vi "Driver_Event.vi"(0 "Data":variant, 2 "Event":T1, 11 "Error In":errorcluster, 13 "Event Operation":T2) -> (4 "Event Ref":refnum<user-event>, 15 "Error Out":errorcluster)   [LabVIEW 2026, in "Core.lvlib"]
doc: "Event driver for all the events in the project."
uses:
  Core.lvlib
  TypeDefs/Enum_Event_Options.ctl
  TypeDefs/Enum_Events.ctl
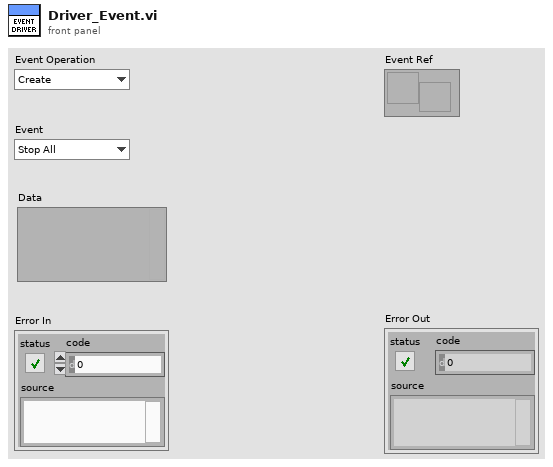
[diagram p1: front panel]
types:
  T1 = typedef "Core.lvlib/Enum_Events.ctl" = enum16{"Stop All", "Stop SubVI", "Update Object"}
  T2 = typedef "Core.lvlib/Enum_Event_Options.ctl" = enum16{"Create", "Generate", "Event Ref", "Destroy"}
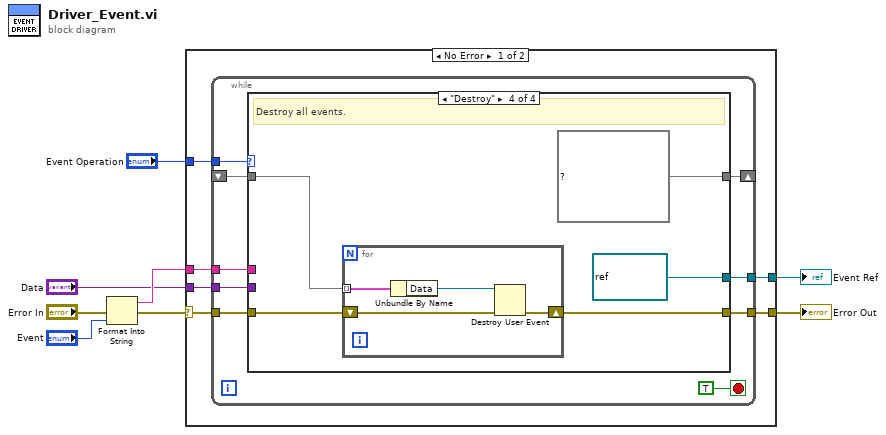
[diagram p0: block diagram]
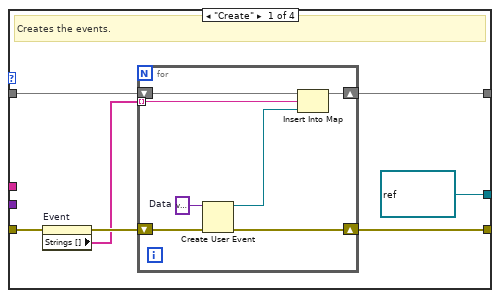
[diagram p2: hidden frame]
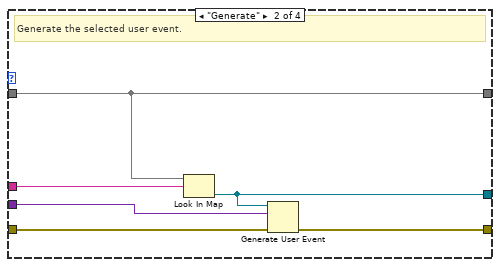
[diagram p3: hidden frame]
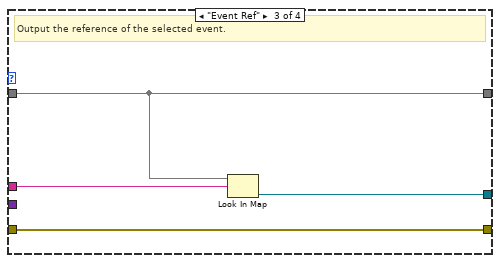
[diagram p4: hidden frame]
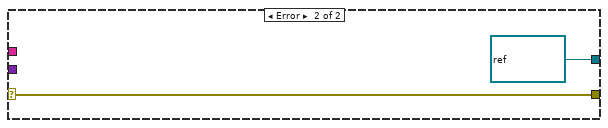
[diagram p5: hidden frame]
diagram:
  n1 = Format Into String(error in="Error In", "Event") -> (resulting string=w3:string, error out=w5:errorcluster)  [unwired: 2 in]
  n2 = case shown="No Error" w5 {
    selector: w5 -> [w13 w58]
    tunnel: [w12 w58] -> w8
    tunnel: "Event Operation" -> [w14 _]
    tunnel: w3 -> [w11 _]
    tunnel: "Data" -> [w10 _]
    tunnel: [w9 refnum<user-event> refnum ("Variant")] -> w1
    frame No Error {
      n3 = while {
        tunnel: w14 -> [w22]
        shift-right: [w17] -> _
        shift-left: _ -> [w18]
        tunnel: w11 -> [w19]
        tunnel: w10 -> [w16]
        tunnel: [w15] -> w9
        tunnel: w13 -> [w20]
        tunnel: [w21] -> w12
        stop <- TRUE stop-if-true
        n4 = case shown="\"Destroy\"" w22 {
          tunnel: [w29 w40 w45 w50] -> w21
          tunnel: w20 -> [w30 w41 w45 w51]
          tunnel: w19 -> [_ w43 w44 _]
          tunnel: w18 -> [w28 w39 w47 w52]
          tunnel: [w27 w39 w47 map{string, refnum<user-event>} {} ("map out")] -> w17
          tunnel: w16 -> [_ w42 _ _]
          tunnel: [refnum<user-event> refnum ("Data") w38 w46 refnum<user-event> refnum ("Data")] -> w15
          frame "Create" {
            # "Creates the events."
            n5 = property on="Event" class="Enum (strict)"(error in=w30) -> (error out=w26:errorcluster, "Strings []"=w25:string[])  [unwired: 1 in, 1 out]
            n6 = for {
              shift-right: [w35] -> w29
              shift-left: w26 -> [w37]
              tunnel: w25 -> [w34] mode=indexing
              shift-right: [w36] -> w27
              shift-left: w28 -> [w31]
              w33 = variant  # Data
              n7 = Create User Event(user event datatype=w33, error in=w37) -> (user event=w32:refnum<user-event>, error out=w35:errorcluster)
              n8 = Insert Into Map(map in=w31, key=w34, value=w32) -> (map out=w36:map{string, refnum<user-event>})  [unwired: 2 out]
            }
          }
          frame "Generate" {
            # "Generate the selected user event."
            n9 = Look In Map(map=w39, key=w43) -> (value=w38:refnum<user-event>)  [unwired: 1 in, 1 out]
            n10 = Generate User Event(user event=w38, event data cluster=w42, error in=w41) -> (error out=w40:errorcluster)  [unwired: 1 in, 1 out]
          }
          frame "Event Ref" {
            # "Output the reference of the selected event."
            n11 = Look In Map(map=w47, key=w44) -> (value=w46:refnum<user-event>)  [unwired: 1 in, 1 out]
          }
          frame "Destroy" {
            # "Destroy all events."
            n12 = for {
              shift-right: [w54] -> w50
              shift-left: w51 -> [w56]
              tunnel: w52 -> [w55] mode=indexing
              n13 = Unbundle By Name(w55) -> ("Data"=w53:refnum<user-event>)
              n14 = Destroy User Event(user event=w53, error in=w56) -> (error out=w54:errorcluster)
            }
          }
        }
      }
    }
    frame Error {
    }
  }
  "Error Out" <- w8
  "Event Ref" <- w1
